vi "Measurement Logic.vi"(8 "error in":errorcluster, 9 "measurement configuration":T2={"double in"=1.2, "Input Terminal Name"=""}, 10 "measure call context in":refnum<class "Measure Call Context.lvclass">) -> (0 "error out":errorcluster, 1 "measurement results":T1, 2 "measure call context out":refnum<class "Measure Call Context.lvclass">)   [LabVIEW 2025, in "Daqmx-Display.lvclass"]
doc: "Contains the core logic for executing the measurement."
uses:
  Daqmx-Display.lvclass
  <vilib>/Plug-In SDKs/Measurements/Measure Call Context/Measure Call Context.lvclass
  Measurement Configuration.ctl
  Measurement Results.ctl
  <vilib>/DAQmx/read.llb/DAQmx Read (Digital 1D Bool 1Chan 1Samp).vi
  <vilib>/DAQmx/create/channels.llb/DAQmx Create Channel (DI-Digital Input).vi
  <vilib>/DAQmx/miscellaneous.llb/DAQmx Fill In Error Info.vi
  <extravilib>/ChannelInstances/Event Messenger-bool/Instantiate.vi
panel:
  out "stop":bool
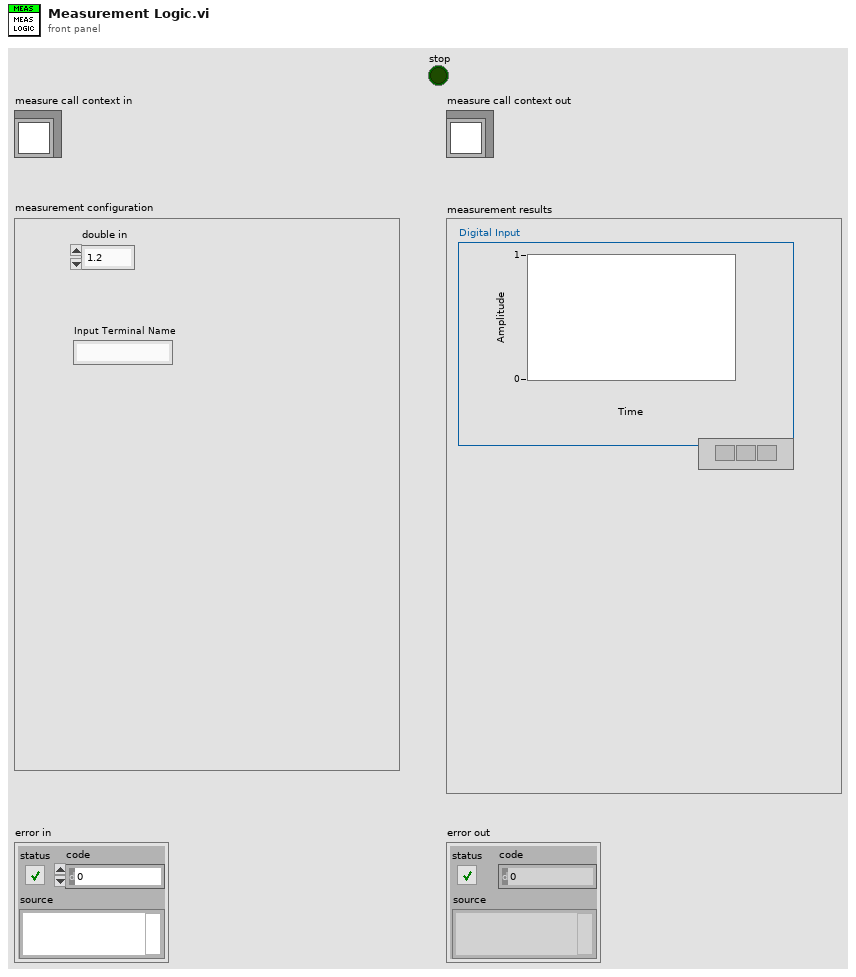
[diagram p1: front panel]
types:
  T1 = typedef "Daqmx-Display.lvclass/Measurement Results.ctl" = cluster{"Digital Input":u32[]}
  T2 = typedef "Daqmx-Display.lvclass/Measurement Configuration.ctl" = cluster{"double in":dbl, "Input Terminal Name":string}
  T3 = typedef "Event Messenger-bool.lvlib/))Channel.ctl" = refnum<queue>
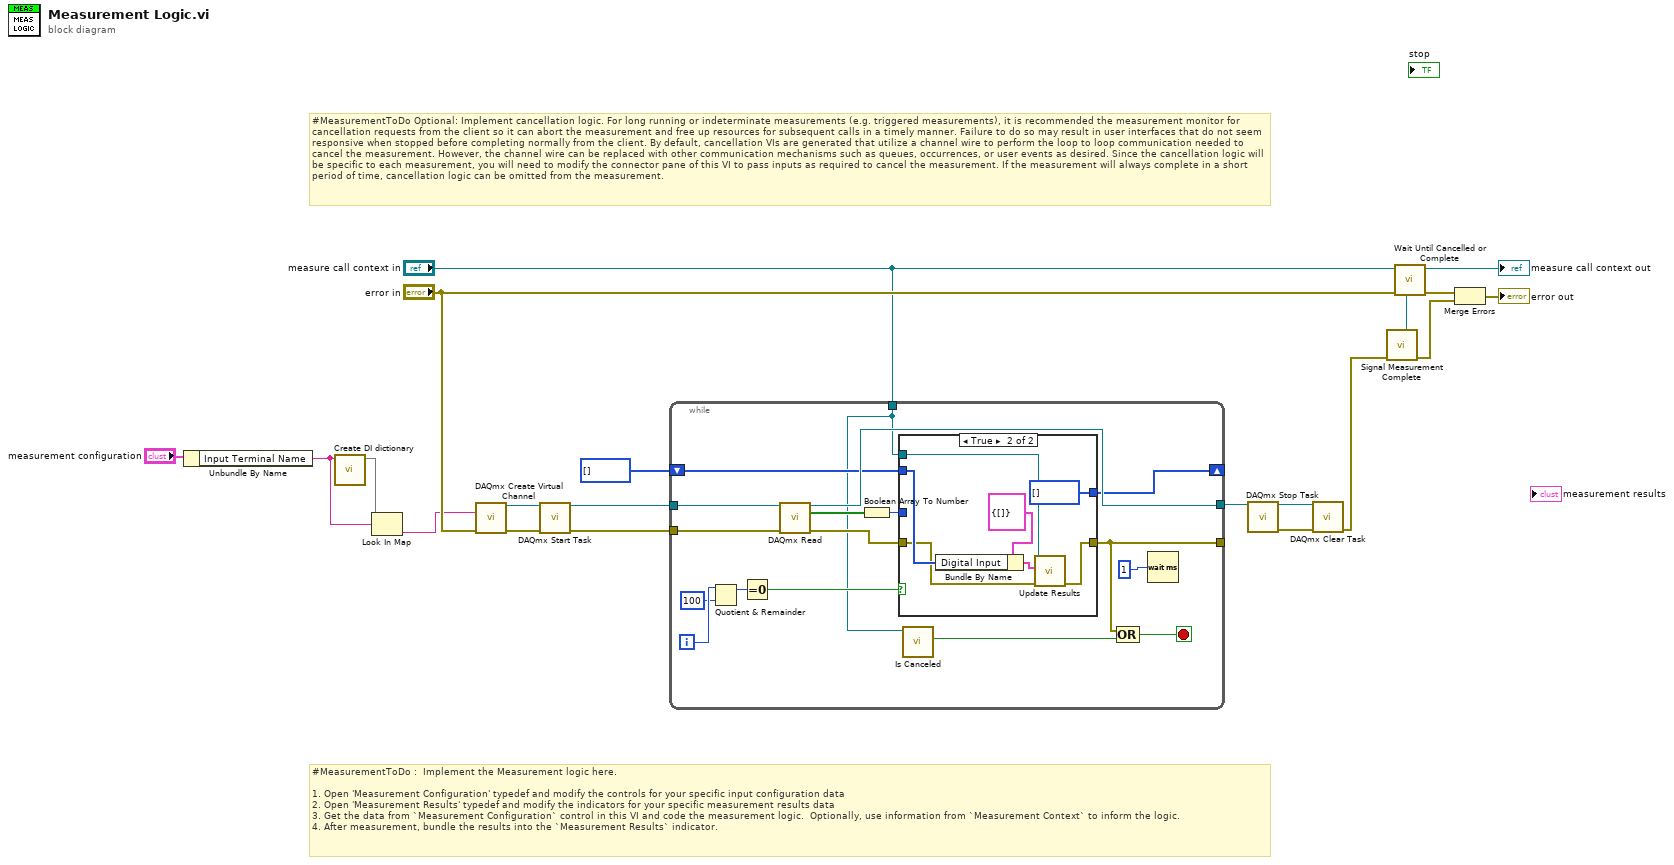
[diagram p0: block diagram]
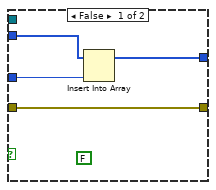
[diagram p2: hidden frame]
diagram:
  # "#MeasurementToDo Optional: Implement cancellation logic. For long running or indeterminate measurements (e.g. triggered measurements), it is recommended the measurement monitor for cancellation requests from the client so it can abort the measurement and free up resources for subsequent calls in a timely manner. Failure to do so may result in user interfaces that do not seem responsive when stopped before completing normally from the client. By default, cancellation VIs are generated that utilize a channel wire to perform the loop to loop communication needed to cancel the measurement. However, the channel wire can be replaced with other communication mechanisms such as queues, occurrences, or user events as desired. Since the cancellation logic will be specific to each measurement, you will need to modify the connector pane of this VI to pass inputs as required to cancel the measurement. If the measurement will always complete in a short period of time, cancellation logic can be omitted from the measurement."
  # "#MeasurementToDo :  Implement the Measurement logic here.\n\n1. Open 'Measurement Configuration' typedef and modify the controls for your specific input configuration data\n2. Open 'Measurement Results' typedef and modify the indicators for your specific measurement results data\n3. Get the data from `Measurement Configuration` control in this VI and code the measurement logic.  Optionally, use information from `Measurement Context` to inform the logic.\n4. After measurement, bundle the results into the `Measurement Results` indicator."
  n1 = Unbundle By Name("measurement configuration") -> ("Input Terminal Name"=w2:string)
  n2 = call "Create DI dictionary.vi"("PFI Input"=w2) -> ("map"=w3:map{string, string})  [unwired: 10 in]
  n3 = Look In Map(map=w3, key=w2) -> (value=w1:string)  [unwired: 1 in, 1 out]
  n4 = call-poly <vilib>:"DAQmx Create Virtual Channel.vi"("lines"=w1, "error in"="error in") -> ("task out"=w13:refnum<k21>, "error out"=w14:errorcluster)  [unwired: 12 in]
  n5 = call <vilib>:"DAQmx Start Task.vi"("task/channels in"=w13, "error in"=w14) -> ("task out"=w12:refnum<k21>, "error out"=w11:errorcluster)  [unwired: 12 in]
  n6 = while {
    tunnel: [w37] -> w6
    tunnel: w12 -> [w36]
    shift-right: [w28] -> _
    shift-left: u32[] [] -> [w27]
    tunnel: w11 -> [w25]
    tunnel: "measure call context in" -> [w22]
    tunnel: [w21] -> _
    i -> [w34]
    stop <- w26 stop-if-true
    n7 = Quotient & Remainder(x=w34, y=100) -> (x-y*floor(x/y)=w32:i32)  [unwired: 1 out]
    n8 = Equal To 0?(x=w32) -> (x = 0?=w31:bool)
    n9 = call-poly <vilib>:"DAQmx Read.vi"("task/channels in"=w36, "error in"=w25) -> ("task out"=w37:refnum<k21>, "data"=w30:bool[], "error out"=w24:errorcluster)  [unwired: 11 in]
    n10 = Boolean Array To Number(Boolean array=w30) -> (number=w29:u32)
    n11 = case shown="True" w31 {
      tunnel: w29 -> [w40 _]
      tunnel: w27 -> [w41 w46]
      tunnel: [w39 u32[] []] -> w28
      tunnel: w24 -> [w38 w43]
      tunnel: [w38 w42] -> w21
      tunnel: w22 -> [_ w45]
      frame False {
        (unwired) FALSE ("is canceled?")
        n12 = Insert Into Array(array=w41, new element=w40) -> (w39:u32[])  [unwired: 1 in]
      }
      frame True {
        n13 = Bundle By Name(cluster=T1 {"Digital Input"=[]} ("Measurement Results"), "Digital Input"=w46) -> (w44:T1)
        n14 = call <vilib>:"Update Results.vi"("error in"=w43, "measurement results"=w44, "measure call context in"=w45) -> ("error out"=w42:errorcluster)  [unwired: 7 in, 1 out]
      }
    }
    n15 = call <vilib>:"Is Canceled.vi"("measure call context in"=w22) -> ("is canceled?"=w23:bool)  [unwired: 8 in, 2 out]
    n16 = Compound Arithmetic op=OR(w21, w23) -> (w26:bool)
    n17 = Wait (ms)(milliseconds to wait=u32 1 ("Loop Time (ms)")) -> ()  [unwired: 1 out]
  }
  n18 = call <vilib>:"DAQmx Stop Task.vi"("task/channels in"=w6) -> ("task out"=w8:refnum<k21>, "error out"=w7:errorcluster)  [unwired: 13 in]
  n19 = call <vilib>:"DAQmx Clear Task.vi"("task in"=w8, "error in"=w7) -> ("error out"=w5:errorcluster)  [unwired: 13 in]
  n20 = call "Signal Measurement Complete.vi"("error in (no error)"=w5) -> ("error out"=w18:errorcluster, "done channel"=w19:T3)  [unwired: 9 in]
  n21 = call "Wait Until Cancelled or Complete.vi"("done channel"=w19, "error in (no error)"="error in", "measure call context in"="measure call context in") -> ("error out"=w17:errorcluster, "measure call context out"=→"measure call context out":refnum<class "Measure Call Context.lvclass">)  [unwired: 7 in]
  n22 = Merge Errors(w17, w18) -> (→"error out":errorcluster)
